vi "Append Table (double).vi"(0 "Document in":refnum<class "Document.lvclass">, 1 "Style":T1={"Name"="Default", "Font"={"Name"="Calibri", "Size"=12, "Bold"=FALSE, "Italic"=FALSE, "Underline"=18, "Strike"=FALSE, "Color"=0, "Alignment"=1}} {"Font"."Alignment" items=["LEFT"=1, "CENTER"=2, "RIGHT"=3, "BOTH"=4, "MEDIUM_KASHIDA"=5, "DISTRIBUTE"=6, "NUM_TAB"=7, "HIGH_KASHIDA"=8, "LOW_KASHIDA"=9, "THAI_DISTRIBUTE"=10]; "Font"."Underline" items=["Single"=1, "Words"=2, "Double"=3, "Thick"=4, "Dotted"=5, "DottedHeavy"=6, "Dash"=7, "DashedHeavy"=8, "DashLong"=9, "DashLongHeavy"=10, "DotDash"=11, "DashDotHeavy"=12, "DotDotDash"=13, "DashDotDotHeavy"=14, "Wave"=15, "WavyHeavy"=16, "WavyDouble"=17, "None"=18]}, 5 "Table":dbl[][](array[numeric]), 7 "Column Headers":string[](array[string]), 9 "Row Headers":string[](array[string]), 11 "error in (no error)":errorcluster) -> (4 "Document out":refnum<class "Document.lvclass">, 15 "error out":errorcluster)   [LabVIEW 2017, in "LabVIEW NPOI.lvlib" / "Document.lvclass"]
doc: "Appends the wire <b>Table</b> as 2D array of doubles to the <b>Document</b> as a table."
uses:
  Document.lvclass
  Styles/Style--cluster.ctl
  Styles/Font--cluster.ctl
  Styles/Underline--ring.ctl
  Styles/Alignment--ring.ctl
  Styles/Styles.lvlib
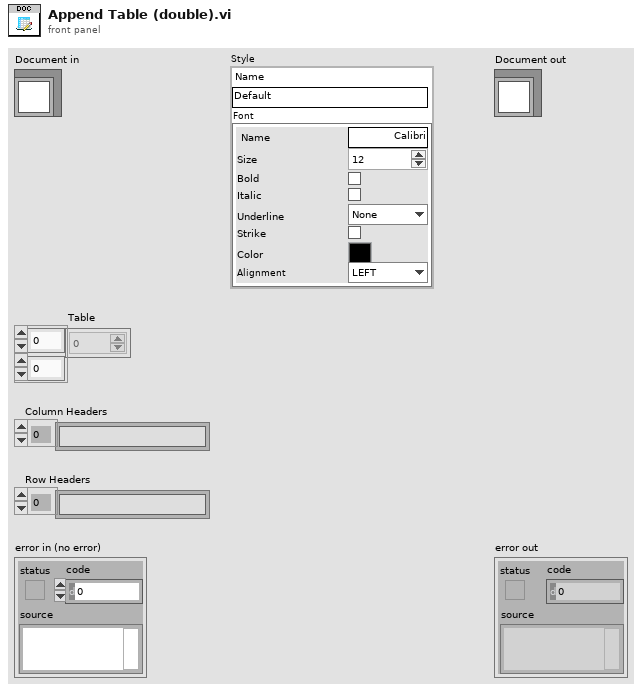
[diagram p1: front panel]
types:
  T1 = typedef "Styles.lvlib/Style--cluster.ctl" = cluster{"Name":string, "Font":T2}
  T2 = typedef "Styles.lvlib/Font--cluster.ctl" = cluster{"Name":string, "Size":i32, "Bold":bool, "Italic":bool, "Underline":T3, "Strike":bool, "Color":u32, "Alignment":T4}
  T3 = typedef "Styles.lvlib/Underline--ring.ctl" = i32
  T4 = typedef "Styles.lvlib/Alignment--ring.ctl" = i32
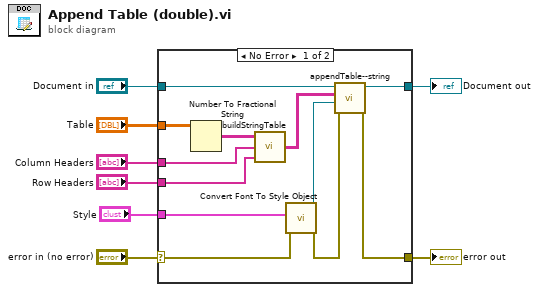
[diagram p0: block diagram]
diagram:
  n1 = case shown="No Error" "error in (no error)" {
    selector: "error in (no error)" -> [w19 w22]
    tunnel: [w14 w22] -> w7
    tunnel: [w15 w21] -> w5
    tunnel: "Document in" -> [w16 w21]
    tunnel: "Table" -> [w10 _]
    tunnel: "Style" -> [w20 _]
    tunnel: "Column Headers" -> [w18 _]
    tunnel: "Row Headers" -> [w17 _]
    frame No Error {
      n2 = Number To Fractional String(number=w10) -> (F-format string=w9:string[][])  [unwired: 3 in]
      n3 = call "buildStringTable.vi"("column headers"=w17, "row headers"=w18, "text data"=w9) -> ("output table"=w11:string[][])
      n4 = call "Convert Font To Style Object.vi"("error in (no error)"=w19, "Style"=w20) -> ("error out"=w12:errorcluster, "Style Object"=w13:refnum<class "Style.lvclass">)  [unwired: 8 in]
      n5 = call-dynamic "appendTable--string.vi"("error in (no error)"=w12, "Font"=w13, "Table"=w11, "Document in"=w16) -> ("error out"=w14:errorcluster, "Document out"=w15:refnum<class "Document.lvclass">)  [unwired: 6 in]
    }
    frame Error {
    }
  }
  "error out" <- w7
  "Document out" <- w5
